vi "CPU_MEM_read_mem.vi"(11 "address":u16 format="%04x") -> (3 "value out":u8 format="%02x")   [LabVIEW 2018]
uses:
  memory/CPU_MEM_references.vi
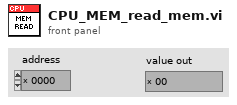
[diagram p1: front panel]
types:
  T1 = enum16{"init", "read DDR", "read PDR", "write DDR", "write PDR"}
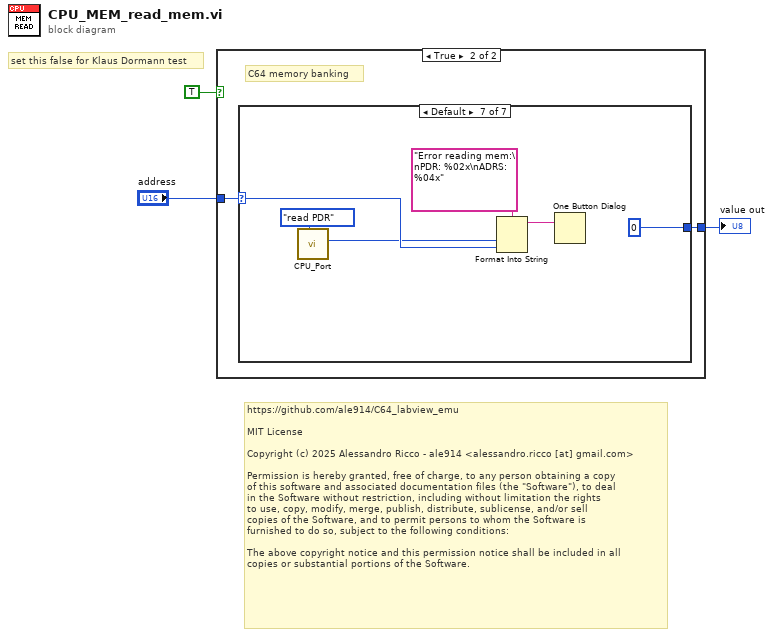
[diagram p0: block diagram]
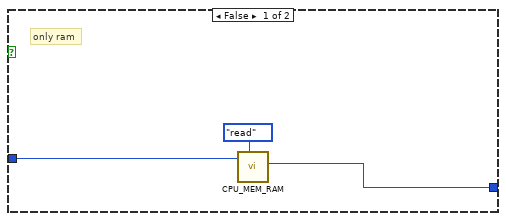
[diagram p2: hidden frame]
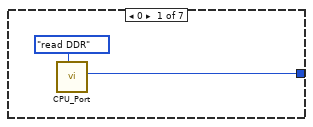
[diagram p3: hidden frame]
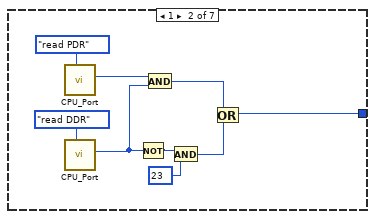
[diagram p4: hidden frame]
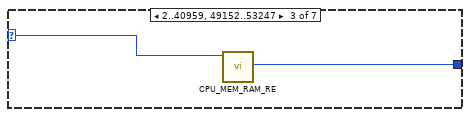
[diagram p5: hidden frame]
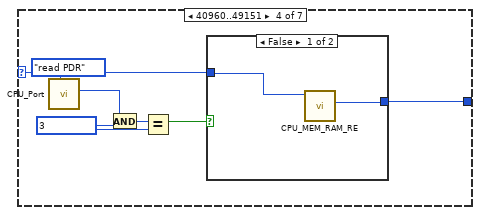
[diagram p6: hidden frame]
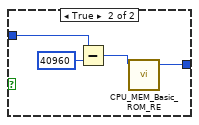
[diagram p7: hidden frame]
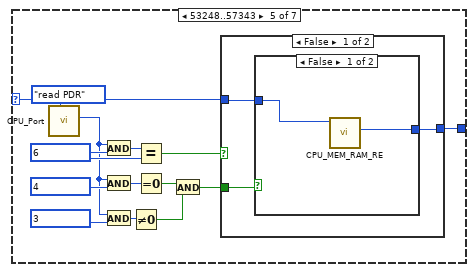
[diagram p8: hidden frame]
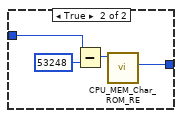
[diagram p9: hidden frame]
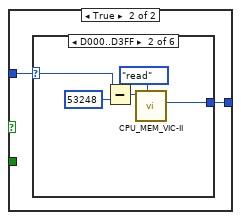
[diagram p10: hidden frame]
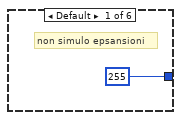
[diagram p11: hidden frame]
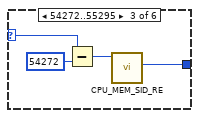
[diagram p12: hidden frame]
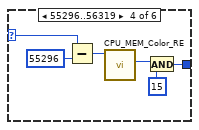
[diagram p13: hidden frame]
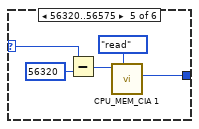
[diagram p14: hidden frame]
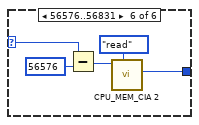
[diagram p15: hidden frame]
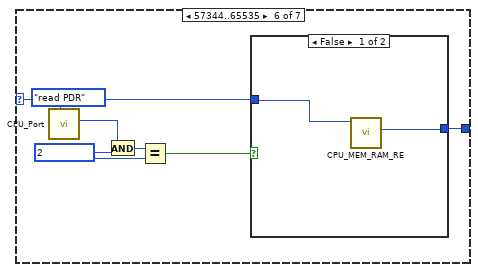
[diagram p16: hidden frame]
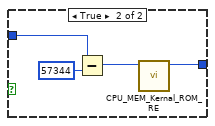
[diagram p17: hidden frame]
diagram:
  # "https://github.com/ale914/C64_labview_emu\n\nMIT License\n\nCopyright (c) 2025 Alessandro Ricco - ale914 <alessandro.ricco [at] gmail.com>\n\nPermission is hereby granted, free of charge, to any person obtaining a copy\nof this software and associated documentation files (the \"Software\"), to deal\nin the Software without restriction, including without limitation the rights\nto use, copy, modify, merge, publish, distribute, sublicense, and/or sell\ncopies of the Software, and to permit persons to whom the Software is\nfurnished to do so, subject to the following conditions:\n\nThe above copyright notice and this permission notice shall be included in all\ncopies or substantial portions of the Software."
  # "set this false for Klaus Dormann test"
  n1 = case shown="True" TRUE {
    tunnel: "address" -> [w5 w8]
    tunnel: [w4 w7] -> w2
    frame False {
      # "only ram"
      n2 = call "CPU_MEM_RAM.vi"("oper"=enum16{"init", "read", "write"}."read", "address"=w5) -> ("value out"=w4:u8)  [unwired: 8 in, 1 out]
    }
    frame True {
      # "C64 memory banking"
      n3 = case shown="Default" w8 {
        selector: w8 -> [_ _ w20 w27 w45 w89 w101]
        tunnel: [w9 w14 w21 w28 w46 w90 u8 0 ("value out")] -> w7
        frame 0 {
          n4 = call "CPU_Port.vi"("oper"=T1."read DDR") -> ("value out"=w9:u8)  [unwired: 10 in]
        }
        frame 1 {
          n5 = call "CPU_Port.vi"("oper"=T1."read PDR") -> ("value out"=w17:u8)  [unwired: 10 in]
          n6 = call "CPU_Port.vi"("oper"=T1."read DDR") -> ("value out"=w16:u8)  [unwired: 10 in]
          n7 = Not(x=w16) -> (.not. x?=w12:u8)
          n8 = And(x=w17, y=w16) -> (x .and. y?=w15:u8)
          n9 = And(x=w12, y=u8 23) -> (x .and. y?=w11:u8)
          n10 = Or(x=w15, y=w11) -> (x .or. y?=w14:u8)
        }
        frame 2..40959, 49152..53247 {
          n11 = call "CPU_MEM_RAM_RE.vi"("address"=w20) -> ("value out"=w21:u8)  [unwired: 10 in]
        }
        frame 40960..49151 {
          w25 = u8 3 ("y")
          n12 = call "CPU_Port.vi"("oper"=T1."read PDR") -> ("value out"=w22:u8)  [unwired: 10 in]
          n13 = And(x=w22, y=w25) -> (x .and. y?=w26:u8)
          n14 = Equal?(x=w26, y=w25) -> (x = y?=w24:bool)
          n15 = case shown="False" w24 {
            tunnel: [w30 w31] -> w28
            tunnel: w27 -> [w29 w34]
            frame False {
              n16 = call "CPU_MEM_RAM_RE.vi"("address"=w29) -> ("value out"=w30:u8)  [unwired: 10 in]
            }
            frame True {
              n17 = Subtract(x=w34, y=u16 40960 ("address")) -> (x-y=w32:u16)
              n18 = call "CPU_MEM_Basic_ROM_RE.vi"("address"=w32) -> ("value out"=w31:u8)  [unwired: 10 in]
            }
          }
        }
        frame 53248..57343 {
          w44 = u8 6 ("y")
          n19 = call "CPU_Port.vi"("oper"=T1."read PDR") -> ("value out"=w35:u8)  [unwired: 10 in]
          n20 = And(x=w35, y=w44) -> (x .and. y?=w48:u8)
          n21 = And(x=w35, y=u8 4) -> (x .and. y?=w42:u8)
          n22 = And(x=w35, y=u8 3) -> (x .and. y?=w39:u8)
          n23 = Not Equal To 0?(x=w39) -> (x != 0?=w38:bool)
          n24 = Equal?(x=w48, y=w44) -> (x = y?=w47:bool)
          n25 = Equal To 0?(x=w42) -> (x = 0?=w41:bool)
          n26 = And(x=w41, y=w38) -> (x .and. y?=w37:bool)
          n27 = case shown="False" w47 {
            tunnel: [w51 w58] -> w46
            tunnel: w45 -> [w50 w59]
            tunnel: w37 -> [w49 _]
            frame False {
              n28 = case shown="False" w49 {
                tunnel: [w53 w57] -> w51
                tunnel: w50 -> [w52 w54]
                frame False {
                  n29 = call "CPU_MEM_RAM_RE.vi"("address"=w52) -> ("value out"=w53:u8)  [unwired: 10 in]
                }
                frame True {
                  n30 = Subtract(x=w54, y=u16 53248 ("address")) -> (x-y=w55:u16)
                  n31 = call "CPU_MEM_Char_ROM_RE.vi"("address"=w55) -> ("value out"=w57:u8)  [unwired: 10 in]
                }
              }
            }
            frame True {
              n32 = case shown="D000..D3FF" w59 {
                selector: w59 -> [_ w64 w67 w74 w79 w84]
                tunnel: [u8 255 ("value out") w65 w69 w70 w80 w85] -> w58
                frame Default {
                  # "non simulo epsansioni"
                }
                frame 53248..54271 {
                  n33 = Subtract(x=w64, y=u16 53248 ("address")) -> (x-y=w61:u16)
                  n34 = call "CPU_MEM_VIC-II.vi"("oper"=enum16{"init", "read", "write"}."read", "address"=w61) -> ("value out"=w65:u8)  [unwired: 8 in, 1 out]
                }
                frame 54272..55295 {
                  n35 = Subtract(x=w67, y=u16 54272 ("address")) -> (x-y=w66:u16)
                  n36 = call "CPU_MEM_SID_RE.vi"("address"=w66) -> ("value out"=w69:u8)  [unwired: 10 in]
                }
                frame 55296..56319 {
                  n37 = Subtract(x=w74, y=u16 55296 ("address")) -> (x-y=w73:u16)
                  n38 = call "CPU_MEM_Color_RE.vi"("address"=w73) -> ("value out"=w72:u8)  [unwired: 10 in]
                  n39 = And(x=w72, y=u8 15 ("address")) -> (x .and. y?=w70:u8)
                }
                frame 56320..56575 {
                  n40 = Subtract(x=w79, y=u16 56320 ("address")) -> (x-y=w76:u16)
                  n41 = call "CPU_MEM_CIA 1.vi"("oper"=enum16{"init", "read", "write"}."read", "address"=w76) -> ("value out"=w80:u8)  [unwired: 8 in, 1 out]
                }
                frame 56576..56831 {
                  n42 = Subtract(x=w84, y=u16 56576 ("address")) -> (x-y=w81:u16)
                  n43 = call "CPU_MEM_CIA 2.vi"("oper"=enum16{"init", "read", "write"}."read", "address"=w81) -> ("value out"=w85:u8)  [unwired: 9 in]
                }
              }
            }
          }
        }
        frame 57344..65535 {
          w88 = u8 2 ("y")
          n44 = call "CPU_Port.vi"("oper"=T1."read PDR") -> ("value out"=w86:u8)  [unwired: 10 in]
          n45 = And(x=w86, y=w88) -> (x .and. y?=w92:u8)
          n46 = Equal?(x=w92, y=w88) -> (x = y?=w91:bool)
          n47 = case shown="False" w91 {
            tunnel: [w94 w95] -> w90
            tunnel: w89 -> [w93 w97]
            frame False {
              n48 = call "CPU_MEM_RAM_RE.vi"("address"=w93) -> ("value out"=w94:u8)  [unwired: 10 in]
            }
            frame True {
              n49 = Subtract(x=w97, y=u16 57344 ("address")) -> (x-y=w96:u16)
              n50 = call "CPU_MEM_Kernal_ROM_RE.vi"("address"=w96) -> ("value out"=w95:u8)  [unwired: 10 in]
            }
          }
        }
        frame Default {
          n51 = call "CPU_Port.vi"("oper"=T1."read PDR") -> ("value out"=w99:u8)  [unwired: 10 in]
          n52 = Format Into String(format string="Error reading mem:\nPDR: %02x\nADRS: %04x", w99, w101) -> (resulting string=w102:string)  [unwired: 2 in, 1 out]
          n53 = One Button Dialog(message=w102) -> ()  [unwired: 1 in, 1 out]
        }
      }
    }
  }
  "value out" <- w2
